vi "Scene_Blit.vi"(0 "Grid":u8[][](array[numeric]), 1 "View":T2={"Hide"=FALSE, "CX"=0, "CY"=0, "ClaudeIdx"=-1, "ClaudeX"=0, "ClaudeY"=0}, 2 "Hud":T1, 3 "Title":T1, 7 "Sprites":cluster{"Pix":u8[][], "Mask":u8[][]}[](array[cluster]), 9 "State":T3={"Tick"=0, "Phase"=0, "PhaseTicks"=0, "Level"=1, "Room"=0, "X10"=0, "Y10"=0, "VY10"=0, "Mode"=0, "Facing"=0, "Run"=0, "Vert"=0, "StandY"=0, "EntryX10"=0, "EntryY10"=0, "EntryMode"=0, "Lives"=4, "Score"=0, "NextLife"=10000, "KeyR"=0, "KeyB"=0, "KeyY"=0, "Torch"=FALSE, "FloorPhase"=0, "Dead"=FALSE, "LevelStart"=FALSE, "Quit"=FALSE, "Sound"=0, "Seed"=12345, "DemoStep"=0, "Tiles"=[], "World"=[], "Enemies"=[], "Highscores"=[], "Name"=[0, 0, 0], "Cursor"=0}, 11 "error in":errorcluster) -> (4 "Picture":u8[][](array[numeric]), 15 "error out":errorcluster)   [LabVIEW 2020, in "GH_Render.lvlib"]
doc: "Builds the WHOLE screen in one raster (rows x width*3 RGB), without any picture drawing: on the title the title image and the overlay; otherwise the HUD image with its values on top of the room raster (Grid, lit or the dark composite), the objects (Room_Blit), the enemies, Claude and the message of the phase."
uses:
  GH_Render.lvlib
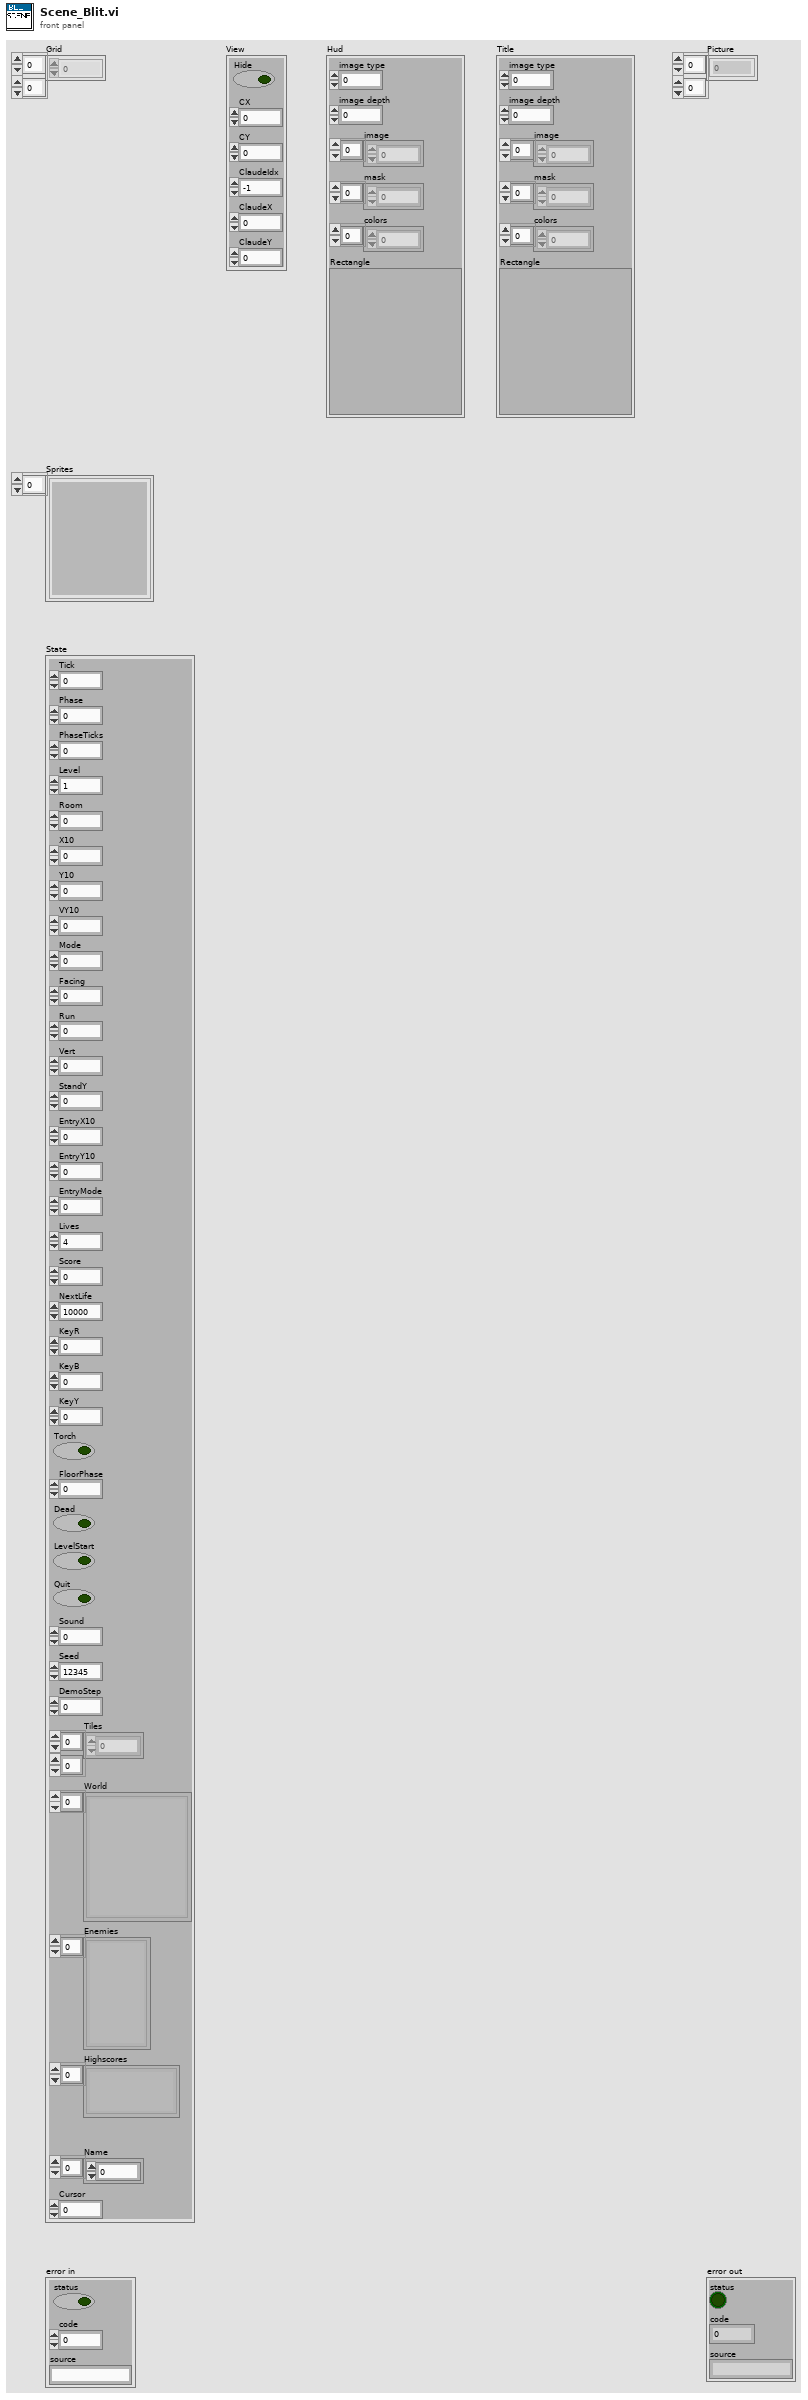
[diagram p1: front panel]
types:
  T1 = cluster{"image type":i32, "image depth":i32, "image":u8[], "mask":u8[], "colors":u32[], "Rectangle":cluster{"left":i16, "top":i16, "right":i16, "bottom":i16}}
  T2 = cluster{"Hide":bool, "CX":i32, "CY":i32, "ClaudeIdx":i32, "ClaudeX":i32, "ClaudeY":i32}
  T3 = cluster{"Tick":u32, "Phase":i32, "PhaseTicks":i32, "Level":i32, "Room":i32, "X10":i32, "Y10":i32, "VY10":i32, "Mode":i32, "Facing":i32, "Run":i32, "Vert":i32, "StandY":i32, "EntryX10":i32, "EntryY10":i32, "EntryMode":i32, "Lives":i32, "Score":i32, "NextLife":i32, "KeyR":i32, "KeyB":i32, "KeyY":i32, "Torch":bool, "FloorPhase":i32, "Dead":bool, "LevelStart":bool, "Quit":bool, "Sound":i32, "Seed":u32, "DemoStep":i32, "Tiles":u8[][], "World":cluster{"ID":string, "Depth":i32, "Column":i32, "Tiles":u8[][]}[], "Enemies":cluster{"Kind":i32, "X10":i32, "Y10":i32, "Dir":i32, "Mode":i32}[], "Highscores":cluster{"Score":i32, "Name":string}[], "Name":i32[], "Cursor":i32}
  T4 = cluster{"left":i16, "top":i16, "right":i16, "bottom":i16}
  T5 = cluster{"Kind":i32, "X10":i32, "Y10":i32, "Dir":i32, "Mode":i32}[]
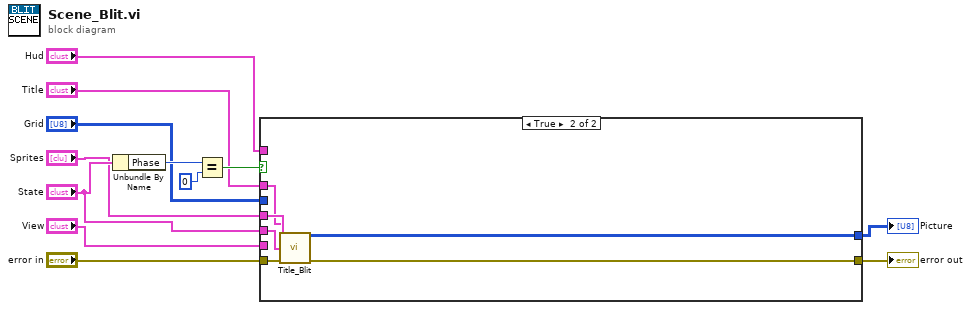
[diagram p0: block diagram]
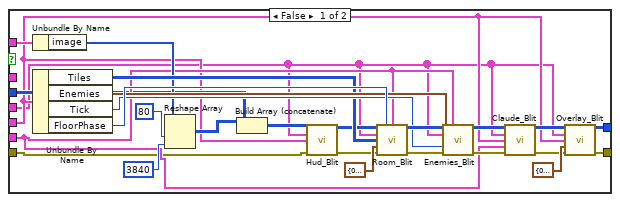
[diagram p2: hidden frame]
diagram:
  n1 = Unbundle By Name("State") -> ("Phase"=w8:i32)
  n2 = Equal?(x=w8, y=0) -> (x = y?=w10:bool)
  n3 = case shown="True" w10 {
    tunnel: "Title" -> [_ w40]
    tunnel: "Sprites" -> [w13 w41]
    tunnel: "State" -> [w14 w42]
    tunnel: "error in" -> [w15 w43]
    tunnel: "Grid" -> [w16 _]
    tunnel: "View" -> [w17 _]
    tunnel: "Hud" -> [w18 _]
    tunnel: [w38 w44] -> w11
    tunnel: [w39 w45] -> w12
    frame False {
      n4 = Unbundle By Name(w18) -> ("image"=w19:u8[])
      n5 = Unbundle By Name(w14) -> ("Tiles"=w26:u8[][], "Enemies"=w27:T5, "Tick"=w28:u32, "FloorPhase"=w29:i32)
      n6 = Reshape Array(w19, 80, 3840) -> (w22:u8[][])
      n7 = Build Array (concatenate)(w22, w16) -> (w23:u8[][])
      n8 = call "Hud_Blit.vi"("Picture"=w23, "Sprites"=w13, "State"=w14, "error in"=w15) -> ("Picture out"=w24:u8[][], "error out"=w25:errorcluster)  [unwired: 10 in]
      n9 = call "Room_Blit.vi"("Picture"=w24, "FloorPhase"=w29, "View"=w17, "Sprites"=w13, "Tiles"=w26, "Region"=T4 {"left"=0, "top"=0, "right"=40, "bottom"=20}, "error in"=w25) -> ("Picture out"=w31:u8[][], "error out"=w32:errorcluster)  [unwired: 7 in]
      n10 = call "Enemies_Blit.vi"("Picture"=w31, "View"=w17, "Sprites"=w13, "Enemies"=w27, "Tick"=w28, "error in"=w32) -> ("Picture out"=w33:u8[][], "error out"=w34:errorcluster)  [unwired: 8 in]
      n11 = call "Claude_Blit.vi"("Picture"=w33, "Sprites"=w13, "State"=w14, "View"=w17, "error in"=w34) -> ("Picture out"=w35:u8[][], "error out"=w36:errorcluster)  [unwired: 9 in]
      n12 = call "Overlay_Blit.vi"("Picture"=w35, "Sprites"=w13, "State"=w14, "Clip"=T4 {"left"=0, "top"=0, "right"=1280, "bottom"=720} ("Whole screen"), "error in"=w36) -> ("Picture out"=w38:u8[][], "error out"=w39:errorcluster)  [unwired: 9 in]
    }
    frame True {
      n13 = call "Title_Blit.vi"("Title"=w40, "Sprites"=w41, "State"=w42, "error in"=w43) -> ("Picture"=w44:u8[][], "error out"=w45:errorcluster)  [unwired: 10 in]
    }
  }
  "Picture" <- w11
  "error out" <- w12
